vi "Main - Call and Monitor TCP Traffic.vi"() -> ()   [LabVIEW 2017, in "Multi-Loop Module Example.lvlib"]
doc: "#### Overview\n\nImplements a TCP server program based on calling `TCP Server Module(Multi-Loop Support).vi`. From the outside, the interaction with this module is identical to that of a standard CSM module. Internally, however, the module's status changes are broadcast via the side loop.\n\n#### Instructions\n\n1. Run this VI.\n2. Run `Simple TCP - Client.vi`.\n3. Modify the string controls on the front panel of both VIs to observe communication logs.\n4. Restart `Simple TCP - Client.vi` as needed to observe reconnection logs.\n\n#### Introduction\n\nWithout using the CSM framework directly, this example implements a TCP server program by calling `TCP Server Module(Multi-Loop Support).vi`. From the outside, the interaction with this module is identical to that of a standard CSM module. Internally, however, the module's status changes are broadcast via the side loop.\n\n#### Steps\n\n- Step1: Initialize UI.\n- Step2: Asynchronously call `TCP Server Module(Multi-Loop Support).vi` to start a CSM module named \"TCPServer\".\n- Step3: Subscribe to the status change events of the TCPServer module.\n- Step4: Modify the string control on the client VI to observe communication logs.\n- Step5: Run `Simple TCP - Client.vi` and click the send button on the VI to send a TCP message to the server.\n- Step6: Any received TCP message is broadcast by the TCPServer as a \"TCP Received\" status change. Therefore, this status can be handled in the status handling event, and this program displays it on the interface.\n- Step7: After modifying the content of the string control and pressing Enter, this program sends it as a TCP message to the Client.\n- Step8: Upon program exit, unsubscribe from the TCPServer module's status change events.\n- Step9: Send the \"Macro: Exit\" message to synchronously exit the TCPServer module."
uses:
  Multi-Loop Module Example.lvlib
  user.lib/_NEVSTOP/Communicable State Machine(CSM)/_Support/Common/Format Timestamp.vi
  user.lib/_NEVSTOP/Communicable State Machine(CSM)/Communicable State Machine.lvlib
panel:
  in  "String":string
  out "String Cache":string
  # "#CSM-Example Overview\n\nImplements a TCP server program based on calling `TCP Server Module(Multi-Loop Support).vi`. From the outside, the interaction with this module is identical to that of a standard CSM module. Internally, however, the module's status changes are broadcast via the side loop."
  # "#CSM-Example Instructions\n\n1. Run this VI.\n2. Run `Simple TCP - Client.vi`.\n3. Modify the string controls on the front panel of both VIs to observe communication logs.\n4. Restart `Simple TCP - Client.vi` as needed to observe reconnection logs."
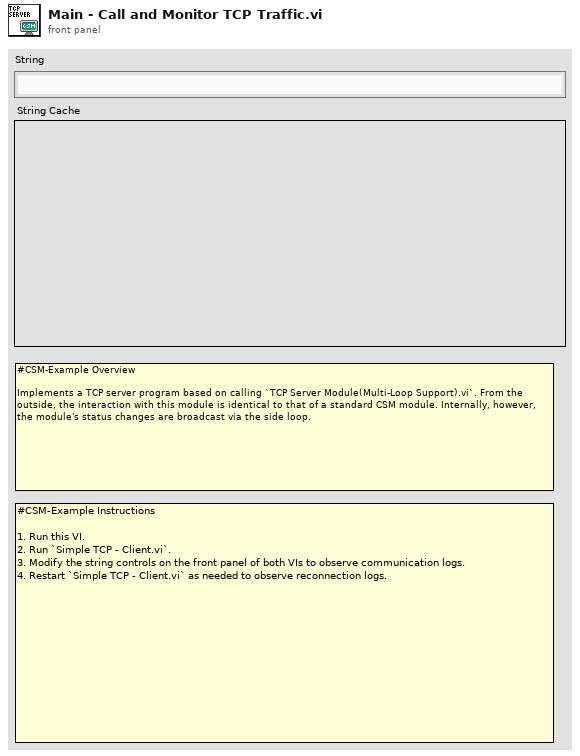
[diagram p1: front panel]
types:
  T1 = cluster{"Status Event":refnum<user-event>, "Interrupt Event":refnum<user-event>}
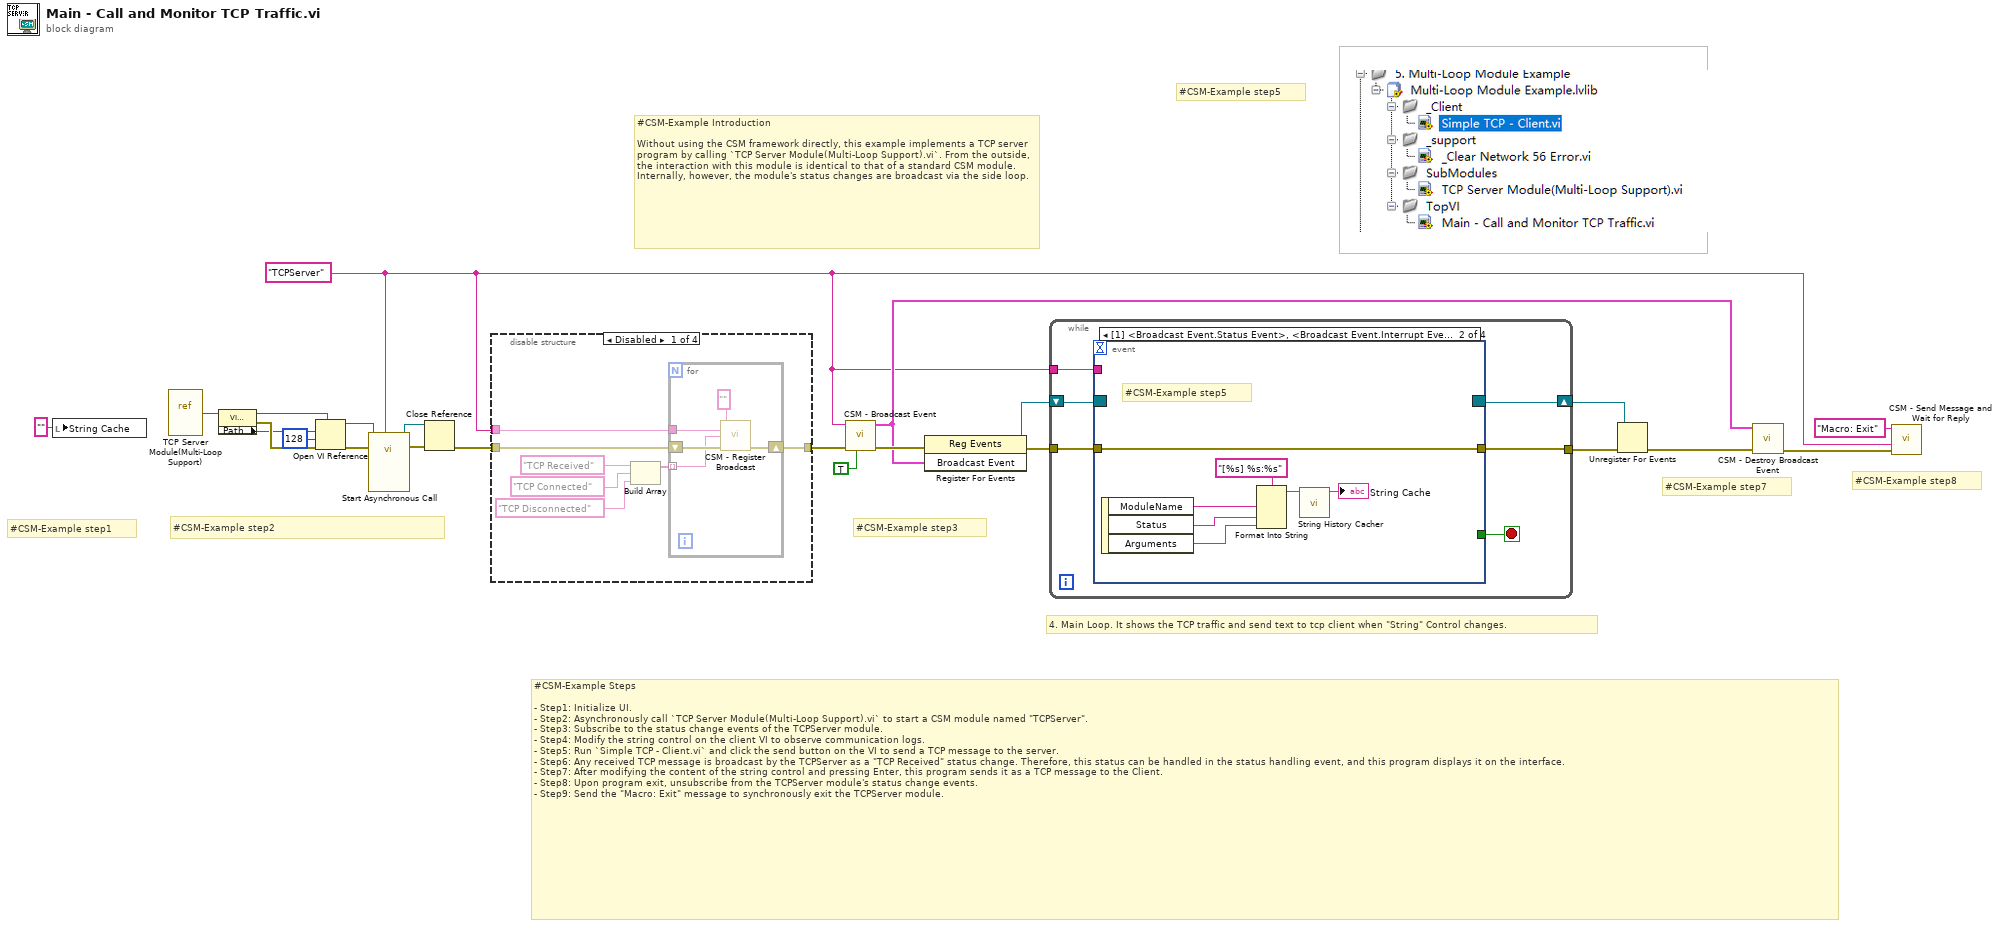
[diagram p0: block diagram]
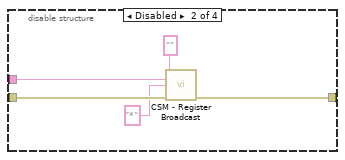
[diagram p2: hidden frame]
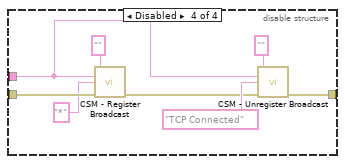
[diagram p4: hidden frame]
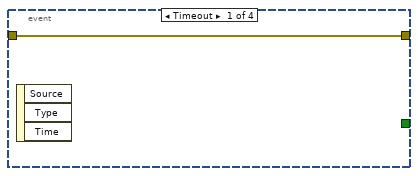
[diagram p5: hidden frame]
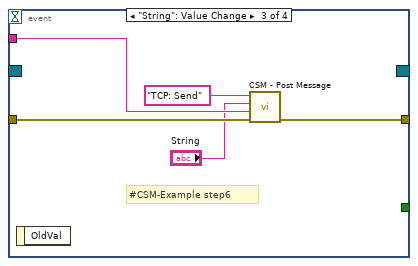
[diagram p6: hidden frame]
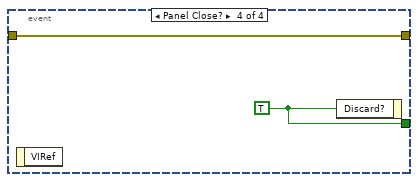
[diagram p7: hidden frame]
diagram:
  w2 = "TCPServer" ("Name (\"\" to Use UUID)")
  # "#CSM-Example step5"
  # "#CSM-Example step8"
  # "#CSM-Example step7"
  # "#CSM-Example step3"
  # "#CSM-Example Steps\n\n- Step1: Initialize UI.\n- Step2: Asynchronously call `TCP Server Module(Multi-Loop Support).vi` to start a CSM module named \"TCPServer\".\n- Step3: Subscribe to the status change events of the TCPServer module.\n- Step4: Modify the string control on the client VI to observe communication logs.\n- Step5: Run `Simple TCP - Client.vi` and click the send button on the VI to send a TCP message to the server.\n- Step6: Any received TCP message is broadcast by the TCPServer as a \"TCP Received\" status change. Therefore, this status can be handled in the status handling event, and this program displays it on the interface.\n- Step7: After modifying the content of the string control and pressing Enter, this program sends it as a TCP message to the Client.\n- Step8: Upon program exit, unsubscribe from the TCPServer module's status change events.\n- Step9: Send the \"Macro: Exit\" message to synchronously exit the TCPServer module."
  # "#CSM-Example Introduction\n\nWithout using the CSM framework directly, this example implements a TCP server program by calling `TCP Server Module(Multi-Loop Support).vi`. From the outside, the interaction with this module is identical to that of a standard CSM module. Internally, however, the module's status changes are broadcast via the side loop."
  # "4. Main Loop. It shows the TCP traffic and send text to tcp client when \"String\" Control changes."
  # "#CSM-Example step2"
  # "#CSM-Example step1"
  n1 = local write "String Cache"("" ("String Cache")) -> ()
  n2 = vi-ref "TCP Server Module(Multi-Loop Support).vi"() -> (w16:refnum<vi>)
  n3 = property class="VI (strict)"(reference=w16) -> (reference out=w20:refnum<vi>, error out=w18:errorcluster, "Path"=w17:path)  [unwired: 1 in]
  n4 = Open VI Reference(type specifier VI Refnum (for type only)=w20, vi path=w17, options=128, error in (no error)=w18) -> (vi reference=w19:refnum<vi>, error out=w15:errorcluster)  [unwired: 2 in]
  n5 = call-by-ref "Start Asynchronous Call"(reference=w19, error in=w15, "Name(\"\" to use uuid)"=w2) -> (reference out=w22:refnum<vi>, error out=w21:errorcluster)  [unwired: 11 in]
  n6 = Close Reference(reference=w22, error in (no error)=w21) -> (error out=w14:errorcluster)
  n7 = disable-structure shown="Disabled" {
    disable-tunnel: w14 -> [w30 w40 w41 w49]
    disable-tunnel: [w29 w38 w41 w43] -> w3
    disable-tunnel: w2 -> [w27 w37 _ w42]
    frame Disabled {
      n8 = Build Array("TCP Received" ("CSM Name"), "TCP Connected" ("CSM Name"), "TCP Disconnected" ("CSM Name")) -> (w26:string[])
      n9 = for {
        tunnel: w26 -> [w32] mode=indexing
        tunnel: w27 -> [w31]
        shift-right: [w34] -> w29
        shift-left: w30 -> [w35]
        n10 = call "CSM - Register Broadcast.vi"("CSM Name(Empty for Broadcast Event)"="" ("CSM Name"), "Source CSM Name (* as Default)"=w31, "Trigger"=w32, "Error In"=w35) -> ("error out"=w34:errorcluster)  [unwired: 10 in, 1 out]
      }
    }
    frame Disabled {
      n11 = call "CSM - Register Broadcast.vi"("CSM Name(Empty for Broadcast Event)"="", "Source CSM Name (* as Default)"=w37, "Trigger"="*" ("CSM Name"), "Error In"=w40) -> ("error out"=w38:errorcluster)  [unwired: 10 in, 1 out]
    }
    frame Enabled {
    }
    frame Disabled {
      n12 = call "CSM - Register Broadcast.vi"("CSM Name(Empty for Broadcast Event)"="" ("CSM Name"), "Source CSM Name (* as Default)"=w42, "Trigger"="*" ("CSM Name"), "Error In"=w49) -> ("error out"=w44:errorcluster)  [unwired: 10 in, 1 out]
      n13 = call "CSM - Unregister Broadcast.vi"("CSM Name(Empty for Broadcast Event)"="" ("CSM Name"), "Source CSM Name (* as Default)"=w42, "Trigger"="TCP Connected" ("CSM Name"), "Error In"=w44) -> ("error out"=w43:errorcluster)  [unwired: 10 in, 1 out]
    }
  }
  n14 = call "CSM - Broadcast Event.vi"("Auto Register? (T)"=TRUE, "Error In"=w3, "CSM Module"=w2) -> ("error out"=w13:errorcluster, "Broadcast Event"=w4:T1)  [unwired: 6 in, 1 out]
  n15 = register-events(error in=w13, w4) -> (reference out=w11:refnum<event-registration>, error out=w12:errorcluster)  [unwired: 1 in]
  n16 = while {
    tunnel: w12 -> [w52]
    tunnel: [w53] -> w7
    tunnel: w2 -> [w51]
    shift-right: [w50] -> w5
    shift-left: w11 -> [w54]
    stop <- w55 stop-if-true
    n17 = event shown="[1] <Broadcast Event.Status Event>, <Broadcast Event.Interrupt Event>: User Event" {
      selector: w54 -> [_ _ _ _]
      dyn-events: [_ _ _ _] -> w50
      timeout: _ -> [_ _ _ _]
      tunnel: [_ _ _ w70] -> w55
      tunnel: [w56 w63 w67 w69] -> w53
      tunnel: w52 -> [w56 w63 w68 w69]
      tunnel: w51 -> [_ _ w66 _]
      event Timeout {
        n18 = event-data() -> ()  [unwired: 1 in, 3 out]
      }
      event User Event {
        # "#CSM-Example step5"
        n19 = event-data() -> ("ModuleName"=w62:string, "Status"=w61:string, "Arguments"=w60:string)  [unwired: 1 in]
        n20 = Format Into String(format string="[%s] %s:%s", w62, w61, w60) -> (resulting string=w58:string)  [unwired: 2 in, 1 out]
        n21 = call "String History Cacher.vi"("String"=w58) -> ("String Cache"=→"String Cache":string)  [unwired: 10 in]
      }
      event "String": Value Change {
        # "#CSM-Example step6"
        n22 = event-data() -> ()  [unwired: 1 in, 1 out]
        n23 = call "CSM - Post Message.vi"("Error In (No Error)"=w68, "Target Module"=w66, "Arguments (\"\")"="String", "State"="TCP: Send") -> ("error out"=w67:errorcluster)  [unwired: 7 in]
      }
      event Panel Close? {
        w70 = TRUE ("Discard?")
        n24 = event-data() -> ()  [unwired: 1 in, 1 out]
        n25 = event-data("Discard?"=w70) -> ()  [unwired: 1 in, 1 out]
      }
    }
  }
  n26 = Unregister For Events(event registration refnum=w5, error in=w7) -> (error out=w6:errorcluster)
  n27 = call "CSM - Destroy Broadcast Event.vi"("Error In"=w6, "Broadcast Event"=w4) -> ("error out"=w10:errorcluster)  [unwired: 9 in]
  n28 = call "CSM - Send Message and Wait for Reply.vi"("Error In (No Error)"=w10, "Target Module"=w2, "State"="Macro: Exit") -> ()  [unwired: 6 in, 3 out]
